vi "Migrate Common Dependencies.vi"(0 "Project path":path, 5 "Measurement path":path, 7 "Dependencies path":path[](array[path]), 11 "error in (no error)":errorcluster) -> (4 "Project reference":refnum<vi>, 6 "MeasurementCore reference":refnum<vi>, 8 "Outside items":string[](array[string]), 15 "error out":errorcluster)   [LabVIEW 2021, in "Multiple Migrator.lvlib"]
uses:
  Multiple Migrator.lvlib
  controls/Library Info.ctl
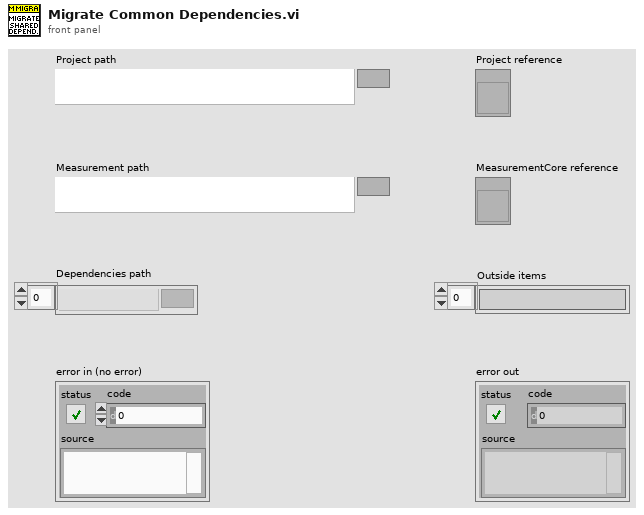
[diagram p1: front panel]
types:
  T1 = typedef "Multiple Migrator.lvlib/Library Info.ctl" = cluster{"Library path":path, "Library name":string}
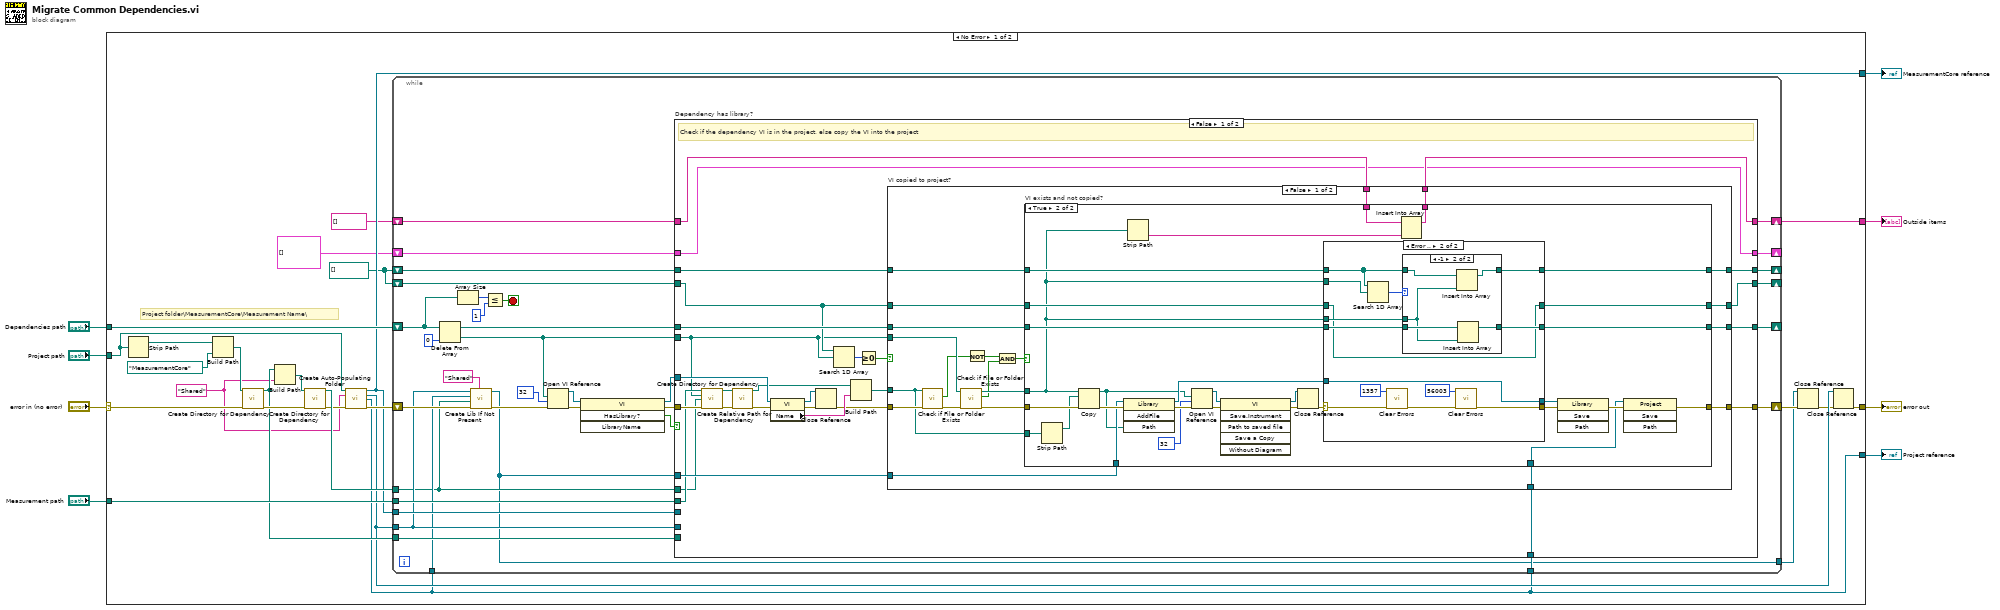
[diagram p0: block diagram]
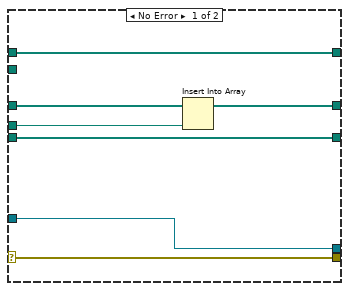
[diagram p3: hidden frame]
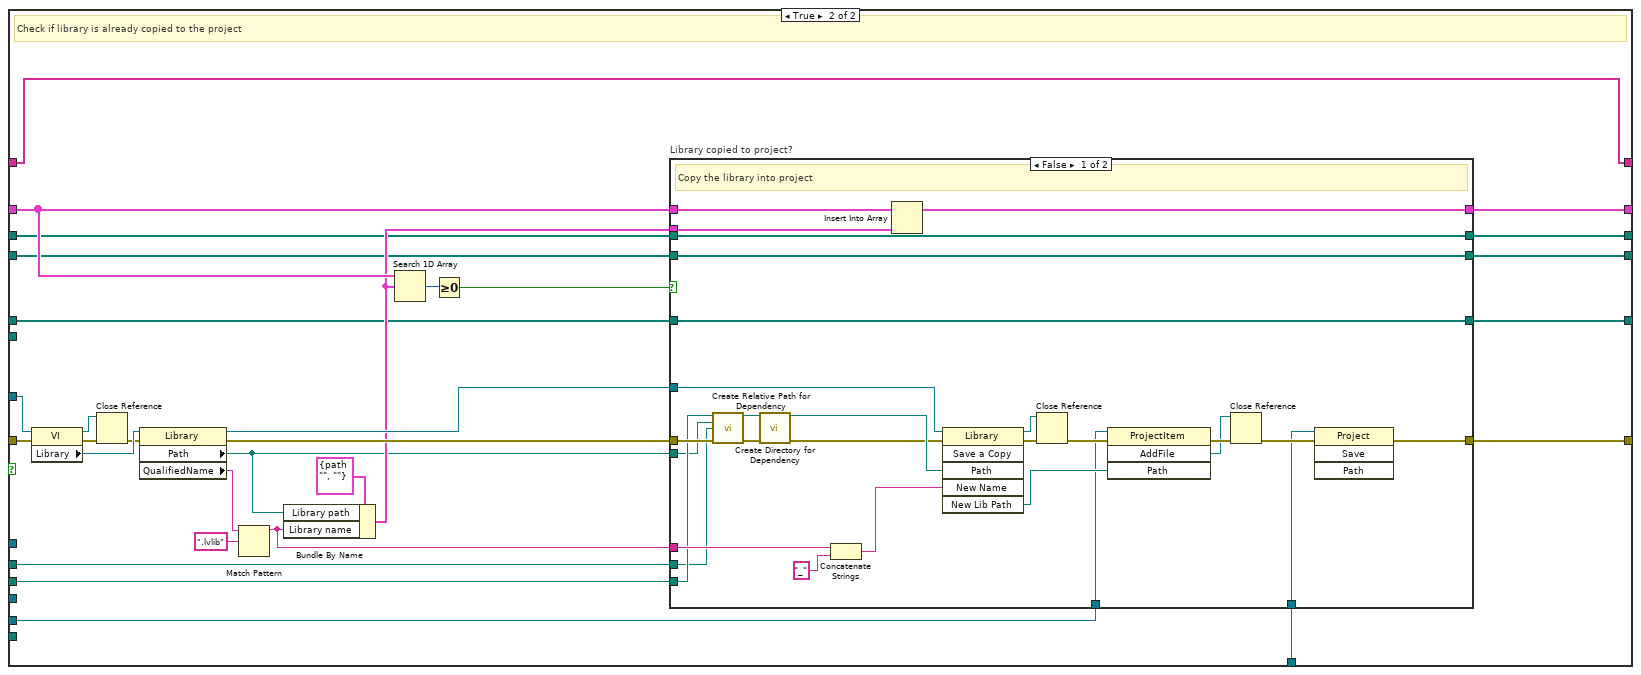
[diagram p6: hidden frame]
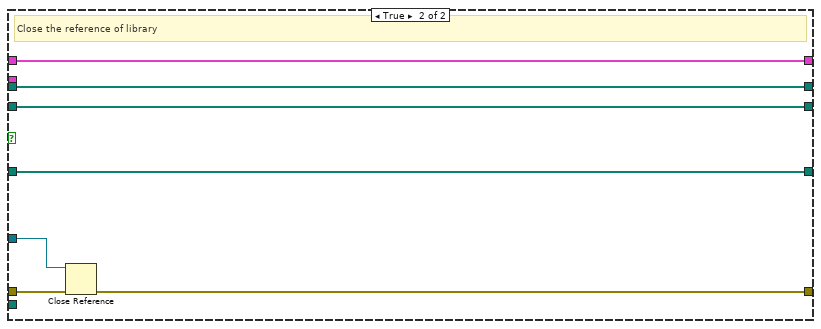
[diagram p7: hidden frame]
diagram:
  n1 = case shown="No Error" "error in (no error)" {
    selector: "error in (no error)" -> [w25 w249]
    tunnel: [w18 w249] -> w7
    tunnel: "Project path" -> [w24 _]
    tunnel: "Measurement path" -> [w29 _]
    tunnel: "Dependencies path" -> [w33 _]
    tunnel: [w20 _] -> w3
    tunnel: [w14 _] -> w2
    tunnel: [w15 _] -> w1
    frame No Error {
      w10 = "Shared"
      w11 = path[] []
      # "Project folder\\MeasurementCore\\Measurement Name\\"
      n2 = Strip Path(path=w24) -> (stripped path=w28:path)  [unwired: 1 out]
      n3 = Build Path(base path=w28, name or relative path=path "MeasurementCore") -> (appended path=w26:path)
      n4 = call "Create Directory for Dependency.vi"("Directory path"=w26, "error in (no error)"=w25) -> ("Directory path out"=w19:path, "error out"=w23:errorcluster)  [unwired: 12 in]
      n5 = Build Path(base path=w19, name or relative path=w10) -> (appended path=w32:path)
      n6 = call "Create Directory for Dependency.vi"("Directory path"=w32, "error in (no error)"=w23) -> ("Directory path out"=w31:path, "error out"=w22:errorcluster)  [unwired: 12 in]
      n7 = call "Create Auto-Populating Folder.vi"("Project path"=w24, "Plug-in name"=w10, "error in (no error)"=w22) -> ("MeasurementCore reference"=w20:refnum<vi>, "Folder reference"=w17:refnum<vi>, "Project reference"=w14:refnum<vi>, "error out"=w21:errorcluster)  [unwired: 9 in]
      n8 = while {
        shift-right: [w55] -> w30
        shift-left: w21 -> [w43]
        shift-right: [w48] -> _
        shift-left: w33 -> [w65]
        tunnel: w31 -> [w39]
        shift-right: [w54] -> _
        shift-left: T1[] [] -> [w57]
        tunnel: w29 -> [w53]
        shift-right: [w50] -> _
        shift-left: w11 -> [w51]
        tunnel: w20 -> [w47]
        tunnel: w19 -> [w46]
        tunnel: w17 -> [w41]
        shift-right: [w44] -> w15
        shift-left: string[] [] -> [w45]
        tunnel: w14 -> [w40]
        tunnel: w14 -> [w38]
        shift-right: [w37] -> _
        shift-left: w11 -> [w36]
        tunnel: [w35] -> w12
        stop <- w64 stop-if-true
        n9 = Delete From Array(array=w65, index=0) -> (deleted portion=w52:path, array with subset deleted=w49:path[])  [unwired: 1 in]
        n10 = Array Size(array=w65) -> (size(s)=w67:i32)
        n11 = call "Create Lib If Not Present.vi"("Plug-in name"="Shared", "error in (no error)"=w43, "DestDirectory"=w39, "ProjectRef"=w40, "VirtualFolderRef"=w41) -> ("error out"=w42:errorcluster, "Library Refnum"=w35:refnum<vi>)  [unwired: 5 in]
        n12 = Less Or Equal?(x=w67, y=1) -> (x <= y?=w64:bool)
        n13 = Open VI Reference(vi path=w52, options=32, error in (no error)=w42) -> (vi reference=w61:refnum<vi>, error out=w63:errorcluster)  [unwired: 3 in]
        n14 = invoke class="VI" method="HasLibrary?"(reference=w61, error in=w63) -> (reference out=w58:refnum<vi>, error out=w59:errorcluster, "Has Library?"=w60:bool)  [unwired: 2 in, 1 out]
        n15 = case "Dependency has library?" shown="False" w60 {
          tunnel: w59 -> [w73 w212]
          tunnel: w58 -> [w94 w213]
          tunnel: w57 -> [w77 w200]
          tunnel: [w89 w201] -> w55
          tunnel: [w77 w199] -> w54
          tunnel: w53 -> [w72 w197]
          tunnel: w39 -> [w70 w195]
          tunnel: w52 -> [w71 _]
          tunnel: w51 -> [w85 w192]
          tunnel: [w81 w191] -> w50
          tunnel: w49 -> [w88 w190]
          tunnel: [w87 w189] -> w48
          tunnel: w47 -> [_ _]
          tunnel: w46 -> [_ _]
          tunnel: w41 -> [_ w188]
          tunnel: w45 -> [w79 w187]
          tunnel: [w78 w187] -> w44
          tunnel: w35 -> [w80 _]
          tunnel: w38 -> [w74 w186]
          tunnel: [w76 w184] -> w37
          tunnel: w36 -> [w75 w185]
          frame False {
            # "Check if the dependency VI is in the project, else copy the VI into the project"
            n16 = call "Create Relative Path for Dependency.vi"("Old Main Path"=w72, "Old Dependency Path"=w71, "New Dir"=w70, "error in (no error)"=w73) -> ("Directory"=w68:path, "error out"=w69:errorcluster)  [unwired: 10 in]
            n17 = call "Create Directory for Dependency.vi"("Directory path"=w68, "error in (no error)"=w69) -> ("Directory path out"=w86:path, "error out"=w95:errorcluster)  [unwired: 12 in]
            n18 = property class="VI"(reference=w94, error in=w95) -> (reference out=w90:refnum<vi>, error out=w93:errorcluster, "Name"=w92:string)
            n19 = Close Reference(reference=w90, error in (no error)=w93) -> (error out=w91:errorcluster)
            n20 = Search 1D Array(1D array=w85, element=w71) -> (index of element=w84:i32)  [unwired: 1 in]
            n21 = Build Path(base path=w86, name or relative path=w92) -> (appended path=w83:path)
            n22 = Greater Or Equal To 0?(x=w84) -> (x >= 0?=w82:bool)
            n23 = case "VI copied to project?" shown="False" w82 {
              tunnel: w91 -> [w116 w183]
              tunnel: w71 -> [w115 _]
              tunnel: [w112 w183] -> w89
              tunnel: w85 -> [w111 w182]
              tunnel: [w110 w182] -> w81
              tunnel: w83 -> [w106 _]
              tunnel: w88 -> [w109 w181]
              tunnel: [w108 w181] -> w87
              tunnel: w79 -> [w101 w180]
              tunnel: [w100 w180] -> w78
              tunnel: w80 -> [w99 _]
              tunnel: [w98 w179] -> w76
              tunnel: w75 -> [w97 w179]
              tunnel: w74 -> [w96 _]
              frame False {
                n24 = call <vilib>:"Check if File or Folder Exists.vi"("error in (no error)"=w116, "path"=w106) -> ("error out"=w107:errorcluster, "file or folder exists?"=w105:bool)  [unwired: 7 in, 1 out]
                n25 = call <vilib>:"Check if File or Folder Exists.vi"("error in (no error)"=w107, "path"=w115) -> ("error out"=w114:errorcluster, "file or folder exists?"=w103:bool, "dup path"=w113:path)  [unwired: 7 in]
                n26 = Not(x=w105) -> (.not. x?=w104:bool)
                n27 = And(x=w104, y=w103) -> (x .and. y?=w102:bool)
                n28 = case "VI exists and not copied?" shown="True" w102 {
                  tunnel: w114 -> [w121 w150]
                  tunnel: w113 -> [_ w130]
                  tunnel: [w121 w132] -> w112
                  tunnel: w111 -> [w120 w149]
                  tunnel: [w120 w148] -> w110
                  tunnel: w106 -> [_ w144]
                  tunnel: w109 -> [w119 w134]
                  tunnel: [w119 w133] -> w108
                  tunnel: w101 -> [w118 w143]
                  tunnel: [w118 w141] -> w100
                  tunnel: w99 -> [_ w140]
                  tunnel: [w117 w139] -> w98
                  tunnel: w97 -> [w117 w138]
                  tunnel: w96 -> [_ w131]
                  frame False {
                  }
                  frame True {
                    n29 = Strip Path(path=w144) -> (stripped path=w146:path)  [unwired: 1 out]
                    n30 = Copy(8:w150, 10:w146, 11:w130) -> (0:w147:errorcluster, 3:w128:path)  [unwired: 2 in, 1 out]
                    n31 = invoke class="Library" method="AddFile"(reference=w140, error in=w147, "Path"=w128) -> (reference out=w137:refnum<vi>, error out=w129:errorcluster)  [unwired: 1 in, 2 out]
                    n32 = Strip Path(path=w130) -> (name=w142:string)  [unwired: 1 out]
                    n33 = Open VI Reference(vi path=w128, options=32, error in (no error)=w129) -> (vi reference=w126:refnum<vi>, error out=w122:errorcluster)  [unwired: 3 in]
                    n34 = invoke class="VI" method="Save.Instrument"(reference=w126, error in=w122) -> (reference out=w124:refnum<vi>, error out=w125:errorcluster)  [unwired: 4 in, 4 out]
                    n35 = Close Reference(reference=w124, error in (no error)=w125) -> (error out=w123:errorcluster)
                    n36 = case shown="Error .." w123 {
                      selector: w123 -> [w152 w171]
                      tunnel: w149 -> [w157 w158]
                      tunnel: [w156 w158] -> w148
                      tunnel: w130 -> [w155 w161]
                      tunnel: [w154 w162] -> w139
                      tunnel: w138 -> [w154 w163]
                      tunnel: [w153 w160] -> w135
                      tunnel: w137 -> [w153 w160]
                      tunnel: [w152 w169] -> w136
                      tunnel: w134 -> [w151 w165]
                      tunnel: [w151 w164] -> w133
                      tunnel: w130 -> [_ w166]
                      frame No Error {
                        n37 = Insert Into Array(array=w157, new element=w155) -> (w156:path[])  [unwired: 1 in]
                      }
                      frame Error {
                        n38 = Search 1D Array(1D array=w163, element=w166) -> (index of element=w159:i32)  [unwired: 1 in]
                        n39 = call <vilib>:"Clear Errors.vi"("error in (no error)"=w171, "specific error code to clear (0: all)"=1357) -> ("error out"=w170:errorcluster)  [unwired: 4 in, 1 out]
                        n40 = case shown="-1" w159 {
                          tunnel: w165 -> [w172 w178]
                          tunnel: [w172 w177] -> w164
                          tunnel: w163 -> [w173 w176]
                          tunnel: [w173 w175] -> w162
                          tunnel: w161 -> [_ w174]
                          frame Default {
                          }
                          frame -1 {
                            n41 = Insert Into Array(array=w176, new element=w174) -> (w175:path[])  [unwired: 1 in]
                            n42 = Insert Into Array(array=w178, new element=w174) -> (w177:path[])  [unwired: 1 in]
                          }
                        }
                        n43 = call <vilib>:"Clear Errors.vi"("error in (no error)"=w170, "specific error code to clear (0: all)"=56003) -> ("error out"=w169:errorcluster)  [unwired: 4 in, 1 out]
                      }
                    }
                    n44 = Insert Into Array(array=w143, new element=w142) -> (w141:string[])  [unwired: 1 in]
                    n45 = invoke class="Library" method="Save"(reference=w135, error in=w136) -> (error out=w145:errorcluster)  [unwired: 2 in, 3 out]
                    n46 = invoke class="Project" method="Save"(reference=w131, error in=w145) -> (error out=w132:errorcluster)  [unwired: 2 in, 3 out]
                  }
                }
              }
              frame True {
              }
            }
          }
          frame True {
            # "Check if library is already copied to the project"
            n47 = property class="VI"(reference=w213, error in=w212) -> (reference out=w203:refnum<vi>, error out=w211:errorcluster, "Library"=w210:refnum<vi>)
            n48 = Close Reference(reference=w203, error in (no error)=w211) -> (error out=w204:errorcluster)
            n49 = property class="Library"(reference=w210, error in=w204) -> (reference out=w202:refnum<vi>, error out=w205:errorcluster, "Path"=w196:path, "QualifiedName"=w206:string)
            n50 = Match Pattern(string=w206, regular expression=".lvlib") -> (before substring=w193:string)  [unwired: 1 in, 3 out]
            n51 = Bundle By Name(cluster=T1 {"Library path"=path "", "Library name"=""} ("Cluster"), "Library path"=w196, "Library name"=w193) -> (w198:T1)
            n52 = Search 1D Array(1D array=w200, element=w198) -> (index of element=w208:i32)  [unwired: 1 in]
            n53 = Greater Or Equal To 0?(x=w208) -> (x >= 0?=w207:bool)
            n54 = case "Library copied to project?" shown="False" w207 {
              tunnel: w205 -> [w218 w247]
              tunnel: w202 -> [w235 w248]
              tunnel: [w222 w246] -> w201
              tunnel: w200 -> [w241 w245]
              tunnel: [w240 w245] -> w199
              tunnel: w198 -> [w239 _]
              tunnel: w197 -> [w217 _]
              tunnel: w196 -> [w216 _]
              tunnel: w195 -> [w215 _]
              tunnel: w193 -> [w225 _]
              tunnel: w192 -> [w232 w244]
              tunnel: [w232 w244] -> w191
              tunnel: [w231 w243] -> w189
              tunnel: w190 -> [w231 w243]
              tunnel: w188 -> [w226 _]
              tunnel: w186 -> [w221 _]
              tunnel: [w220 w242] -> w184
              tunnel: w185 -> [w220 w242]
              frame False {
                # "Copy the library into project"
                n55 = call "Create Relative Path for Dependency.vi"("Old Main Path"=w217, "Old Dependency Path"=w216, "New Dir"=w215, "error in (no error)"=w218) -> ("Directory"=w214:path, "error out"=w219:errorcluster)  [unwired: 10 in]
                n56 = call "Create Directory for Dependency.vi"("Directory path"=w214, "error in (no error)"=w219) -> ("Directory path out"=w236:path, "error out"=w234:errorcluster)  [unwired: 12 in]
                n57 = Concatenate Strings(w225, "_" ("string")) -> (w223:string)
                n58 = Insert Into Array(array=w241, new element=w239) -> (w240:T1[])  [unwired: 1 in]
                n59 = invoke class="Library" method="Save a Copy"(reference=w235, error in=w234, "Path"=w236, "New Name"=w223) -> (reference out=w237:refnum<vi>, error out=w238:errorcluster, "New Lib Path"=w229:path)  [unwired: 2 in, 3 out]
                n60 = Close Reference(reference=w237, error in (no error)=w238) -> (error out=w233:errorcluster)
                n61 = invoke class="ProjectItem" method="AddFile"(reference=w226, error in=w233, "Path"=w229) -> (error out=w230:errorcluster, "AddFile"=w227:refnum<vi>)  [unwired: 1 in, 2 out]
                n62 = Close Reference(reference=w227, error in (no error)=w230) -> (error out=w228:errorcluster)
                n63 = invoke class="Project" method="Save"(reference=w221, error in=w228) -> (error out=w222:errorcluster)  [unwired: 2 in, 3 out]
              }
              frame True {
                # "Close the reference of library"
                n64 = Close Reference(reference=w248, error in (no error)=w247) -> (error out=w246:errorcluster)
              }
            }
          }
        }
      }
      n65 = Close Reference(reference=w12, error in (no error)=w30) -> (error out=w13:errorcluster)
      n66 = Close Reference(reference=w17, error in (no error)=w13) -> (error out=w18:errorcluster)
    }
    frame Error {
    }
  }
  "error out" <- w7
  "MeasurementCore reference" <- w3
  "Project reference" <- w2
  "Outside items" <- w1
